vi "load tags from CSV.vi"(11 "engine ref":refnum<data-value>) -> (2 "load attempted":bool)   [LabVIEW 2013, in "PL Framework Configuration Tool.lvlib" / "EngineTags.lvclass"]
uses:
  EngineTags.lvclass
  Engine Parent/Engine Parent Editor Node.lvclass
  <vilib>/NI/Module Execution Interface/Engine Configuration/engine configuration.lvclass
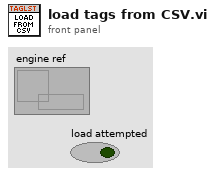
[diagram p1: front panel]
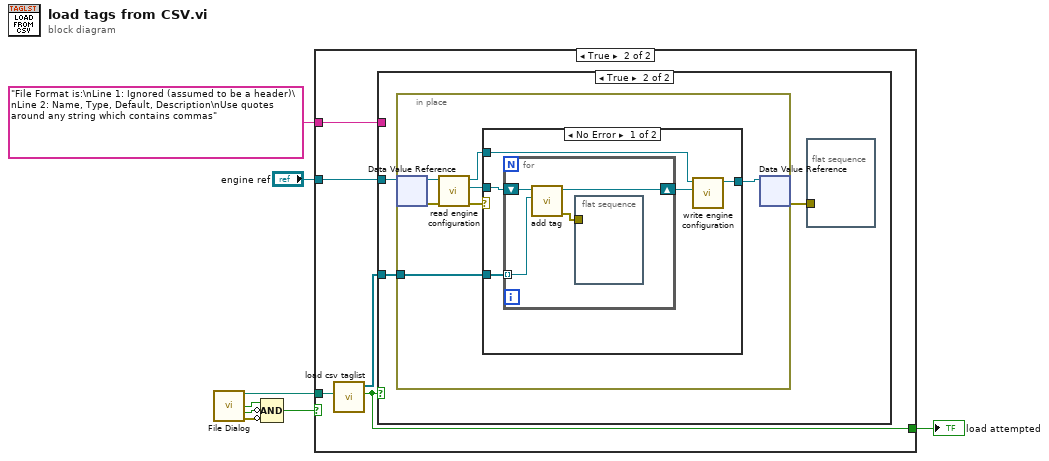
[diagram p0: block diagram]
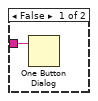
[diagram p3: hidden frame]
diagram:
  n1 = call "File Dialog"() -> ("selected path"=w6:path, "exists"=w5:bool, "cancelled"=w4:bool, "error out"=w3:errorcluster)  [unwired: 12 in]
  n2 = Compound Arithmetic op=AND(w5, invert w4, invert w3) -> (w7:bool)
  n3 = case shown="True" w7 {
    tunnel: w6 -> [_ w12]
    tunnel: [_ w11] -> w8
    tunnel: "File Format is:\nLine 1: Ignored (assumed to be a header)\nLine 2: Name, Type, Default, Description\nUse quotes around any string which contains commas" ("message") -> [_ w10]
    tunnel: "engine ref" -> [_ w9]
    frame False {
    }
    frame True {
      n4 = call "load csv taglist.vi"("cfg file path"=w12) -> ("ok?"=w11:bool, "tags"=w13:refnum<class "tag descriptor.lvclass">[])  [unwired: 9 in]
      n5 = case shown="True" w11 {
        tunnel: w13 -> [_ w17]
        tunnel: w10 -> [w14 _]
        tunnel: w9 -> [_ w15]
        frame False {
          n6 = One Button Dialog(message=w14) -> ()  [unwired: 1 in, 1 out]
        }
        frame True {
          n7 = in-place {
            in-place-border: w17 -> [w24]
            n8 = in-place-dvr #1(w15) -> (w22:refnum<class "Engine Parent Editor Node.lvclass">, w23:errorcluster)
            n9 = call "read engine configuration.vi"("error in"=w23, "Engine Parent Editor Node in"=w22) -> ("error out"=w19:errorcluster, "engine configuration"=w18:refnum<class "engine configuration.lvclass">, "Engine Parent Editor Node out"=w21:refnum<class "Engine Parent Editor Node.lvclass">)  [unwired: 7 in]
            n10 = case shown="No Error" w19 {
              tunnel: w24 -> [w29 _]
              tunnel: w21 -> [w27 w34]
              tunnel: [w26 w34] -> w20
              tunnel: w18 -> [w25 _]
              frame No Error {
                n11 = for {
                  shift-right: [w33] -> w28
                  shift-left: w25 -> [w32]
                  tunnel: w29 -> [w31] mode=indexing
                  n12 = call <vilib>:"add tag.vi"("tag descriptor"=w31, "engine configuration in"=w32) -> ("error out"=w30:errorcluster, "engine configuration out"=w33:refnum<class "engine configuration.lvclass">)  [unwired: 8 in]
                  n13 = flat-sequence {
                    tunnel: w30 -> [_]
                    frame #0 {
                    }
                  }
                }
                n14 = call "write engine configuration.vi"("engine configuration"=w28, "Engine Parent Editor Node in"=w27) -> ("Engine Parent Editor Node out"=w26:refnum<class "Engine Parent Editor Node.lvclass">)  [unwired: 8 in, 1 out]
              }
              frame Error {
              }
            }
            n15 = in-place-dvr #1(w20) -> (w16:errorcluster)  [unwired: 1 out]
          }
          n16 = flat-sequence {
            tunnel: w16 -> [_]
            frame #0 {
            }
          }
        }
      }
    }
  }
  "load attempted" <- w8
